vi "Kill uService.vi"(8 "error in (no error)":errorcluster, 10 "uService":string, 11 "Guardian in":refnum<class "Guardian.lvclass">) -> (0 "error out":errorcluster, 3 "Guardian out":refnum<class "Guardian.lvclass">)   [LabVIEW 2020, in "TALOS.lvlib" / "Guardian.lvlib" / "Guardian.lvclass"]
uses:
  Guardian.lvclass
  Classes/uService List/uService List.lvclass
  builds/Actor Framework PPL/Actor Framework.lvlibp/1abvi3w/vi.lib/ActorFramework/Stop Msg/Stop Msg.lvclass
  Classes/uService List/Set Online Status.vi
  Classes/uService List/Get Queue.vi
  TALOS.lvlib
  C:/LabVIEW Code/TALOS/talos/Ancestor/Ancestor/Ancestor.lvclass
  C:/LabVIEW Code/TALOS/builds/Actor Framework PPL/Actor Framework.lvlibp/1abvi3w/vi.lib/ActorFramework/Actor/Actor.lvclass
  C:/LabVIEW Code/TALOS/talos/Guardian/Guardian/Guardian.lvclass
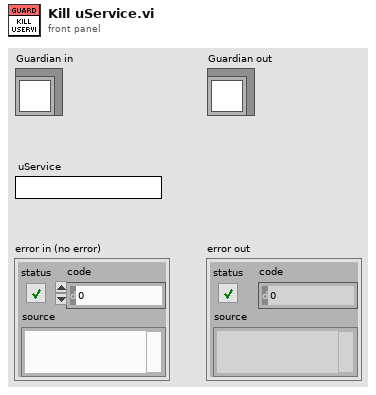
[diagram p1: front panel]
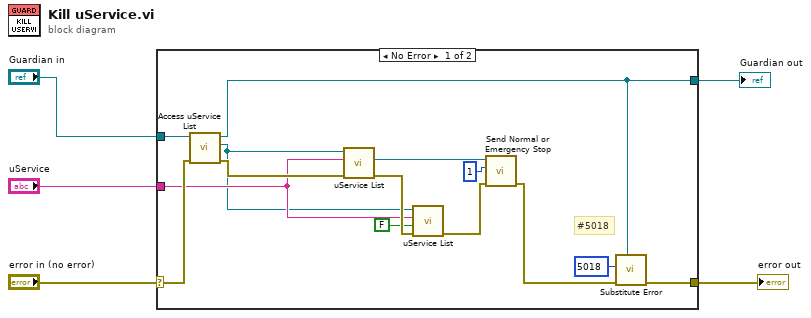
[diagram p0: block diagram]
diagram:
  n1 = case shown="No Error" "error in (no error)" {
    selector: "error in (no error)" -> [w16 w20]
    tunnel: [w8 w20] -> w5
    tunnel: "uService" -> [w15 _]
    tunnel: "Guardian in" -> [w14 w21]
    tunnel: [w7 w21] -> w1
    frame No Error {
      # "#5018"
      n2 = call-dynamic "Access uService List.vi"("error in (no error)"=w16, "Ancestor in"=w14) -> ("error out"=w17:errorcluster, "uService List out"=w13:refnum<class "uService List.lvclass">, "Ancestor out"=w7:refnum<class "Guardian.lvclass">)  [unwired: 7 in]
      n3 = call-poly "uService List.vi"("error in (no error)"=w17, "ID"=w15, "uService List in"=w13) -> ("error out"=w18:errorcluster, "uService Queue"=w12:refnum<class "Message Enqueuer.lvclass">)  [unwired: 6 in, 1 out]
      n4 = call-poly "uService List.vi"("error in (no error)"=w18, "Online"=FALSE, "ID"=w15, "uService List in"=w13) -> ("error out"=w19:errorcluster)  [unwired: 6 in, 1 out]
      n5 = call "Send Normal or Emergency Stop.vi"("error in (no error)"=w19, "final error code"=1, "Message Enqueuer"=w12) -> ("error out"=w9:errorcluster)  [unwired: 8 in]
      n6 = call "Substitute Error.vi"("LabVIEW Object"=w7, "error in (no error)"=w9, "Error Code"=5018) -> ("error out"=w8:errorcluster)  [unwired: 8 in]
    }
    frame Error {
    }
  }
  "error out" <- w5
  "Guardian out" <- w1
